vi "TEST - Get Array Element TD.vi"(8 "error in (no error)":errorcluster) -> (0 "error out":errorcluster, 2 "pass":bool)   [LabVIEW 2020, in "test_openg_array.lvlib"]
uses:
  source/library/Type Descriptor.ctl
  test_openg_array.lvlib
  <userlib>/_OpenG.lib/error/error.llb/openg_error.lvlib
  source/library/openg_variant.lvlib
panel:
  out "Failures":T2(array[cluster])
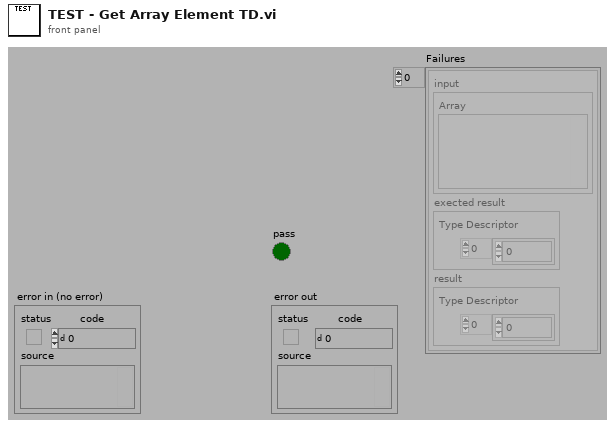
[diagram p1: front panel]
types:
  T1 = typedef "openg_variant.lvlib/Type Descriptor.ctl" = i16[]
  T2 = cluster{"input":cluster{"Array":variant}, "exected result":cluster{"Type Descriptor":T1}, "result":cluster{"Type Descriptor":T1}}[]
  T3 = cluster{"input":cluster{"Array":variant}, "exected result":cluster{"Type Descriptor":T1}, "result":cluster{"Type Descriptor":T1}}
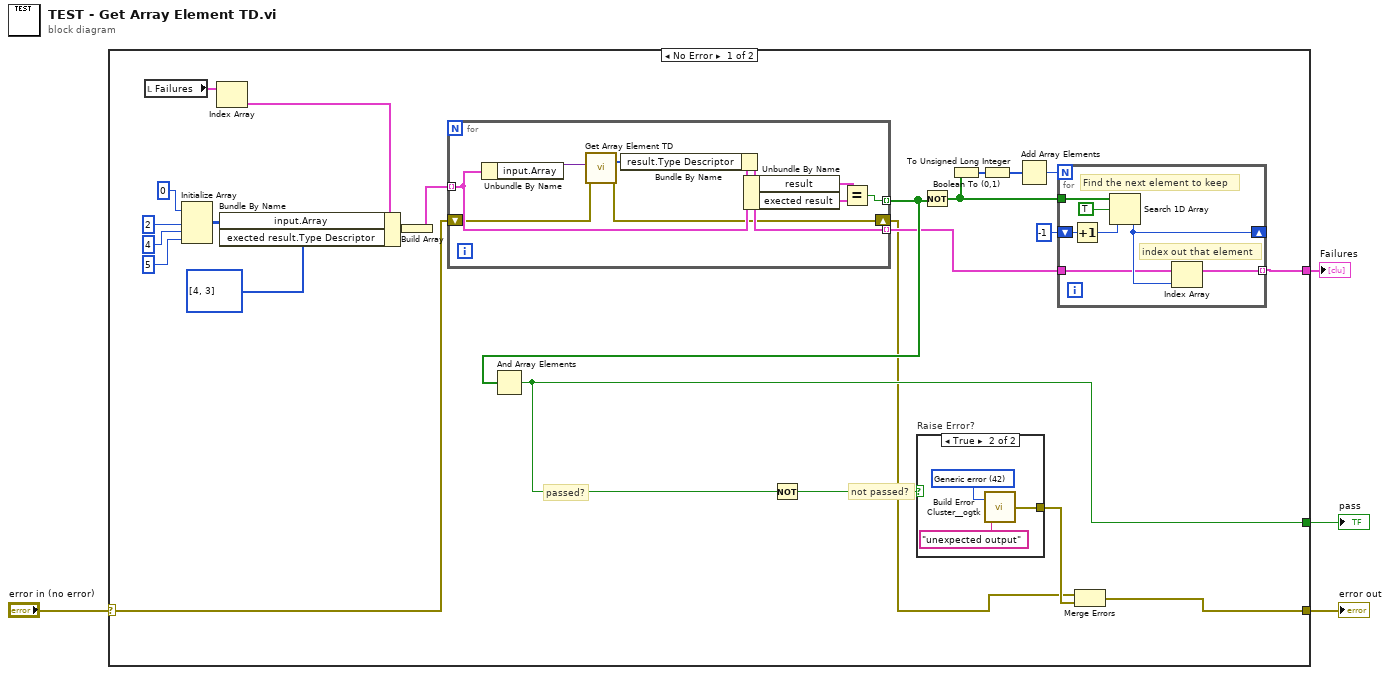
[diagram p0: block diagram]
diagram:
  n1 = case shown="No Error" "error in (no error)" {
    selector: "error in (no error)" -> [w14 w48]
    tunnel: [w25 _] -> w4
    tunnel: [w28 w48] -> w2
    tunnel: [w17 _] -> w1
    frame No Error {
      # "not passed?"
      # "passed?"
      n2 = local read "Failures"() -> (w12:T2)
      n3 = Initialize Array(0, u32 2 ("Numeric"), 4 ("Numeric"), 5 ("Numeric")) -> (w8:i32[][][])
      n4 = Index Array(array=w12) -> (element=w7:T3)  [unwired: 1 in]
      n5 = Bundle By Name(cluster=w7, "input.Array"=w8, "exected result.Type Descriptor"=T1 [4, 3] ("Type Descriptor")) -> (w16:T3)
      n6 = Build Array(w16) -> (w15:T2)
      n7 = for {
        tunnel: w15 -> [w43] mode=indexing
        tunnel: [w44] -> w19 mode=indexing
        tunnel: [w42] -> w18 mode=indexing
        shift-right: [w36] -> w13
        shift-left: w14 -> [w37]
        n8 = Unbundle By Name(w43) -> ("input.Array"=w39:variant)
        n9 = call "Get Array Element TD.vi"("error in (no error)"=w37, "Array"=w39) -> ("error out"=w36:errorcluster, "Type Descriptor"=w38:T1)  [unwired: 8 in]
        n10 = Bundle By Name(cluster=w43, "result.Type Descriptor"=w38) -> (w42:T3)
        n11 = Unbundle By Name(w42) -> ("result"=w41:cluster{"Type Descriptor":T1}, "exected result"=w40:cluster{"Type Descriptor":T1})
        n12 = Equal?(x=w41, y=w40) -> (x = y?=w44:bool)
      }
      n13 = And Array Elements(Boolean array=w19) -> (logical AND=w25:bool)
      n14 = Not(x=w25) -> (.not. x?=w26:bool)
      n15 = case "Raise Error?" shown="True" w26 {
        tunnel: [_ w45] -> w27
        frame False {
        }
        frame True {
          w46 = 42 items=["No error", "Argument error", "Memory is full", "Out of zone", "End of file", "File already open", "Generic file I/O error", "File not found", "File permission error", "Disk is full", "Duplicate path", "Too many files open", "System feature not enabled", "Resource file not found", "Cannot add resource", "Resource not found", "Image not found", "Image memory error", "Pen does not exist", "Config type invalid", "Config token not found", "Config parse error", "Config memory error", "Bad external code format", "Bad external code offset", "External code not present", "Null window", "Destroy window error", "Null menu", "Print aborted", "Bad print record", "Print driver error", "Windows error during printing", "Memory error during printing", "Print dialog error", "Generic print error", "Invalid device refnum", "Device not found", "Device parameter error", "Device unit error", "Cannot open device", "Device call aborted", "Generic error", "Cancelled by user", "Object ID too low", "Object ID too high", "Object not in heap", "Unknown heap", "Unknown object (invalid DefProc)", "Unknown object (DefProc not in table)", "Message out of range", "Invalid (null) method", "Unknown message", "Manager call not supported", "Bad address", "Network operation in progress", "Network operation timed out", "Connection is busy", "Network attribute not supported", "Network error", "Address in use", "System out of memory", "Connection aborted", "Connection refused", "Not connected", "Already connected", "Connection closed", "Initialization error (interapplication manager)", "Bad occurrence", "Wait on unbound occurrence handler", "Occurrence queue overflow", "Datalog type conflict", "Unused", "Unrecognized type (interapplication manager)", "Memory corrupt", "Failed to make temporary DLL", "Old CIN version", "Drag socket not found", "Failed to load drop-object", "Failed to register OLE object", "Failed to release OLE object", "Format specifier type mismatch", "Unknown format specifier", "Too few format specifiers", "Too many format specifiers", "Scan failed", "Newer CIN version", "Error converting to variant", "Runtime menu error", "Password tampered", "Variant attribute not found", "Incompatible variant data type", "Event data is not available", "Event Store is not present", "Occurrence is not found", "Event Queue is not created", "Event info is not available", "Refnum passed is NULL", "Error retrieving Class GUID", "Error retrieving CoClass GUID", "Error retrieving TypeLib GUID.", "Bad built application magic bytes.", "Specific driver is different from the specific driver associated with the Logical Name.", "There is no session opened to the class driver.", "Max Error", "MAX - Error with config objects", "MAX - Error loading configuration", "MAX - Group not supported"]
          n16 = call <userlib>:"Build Error Cluster__ogtk.vi"("String to Prepend to source (\"\")"="unexpected output" ("String to Prepend to source (\"\")"), "code"=w46) -> ("error out"=w45:errorcluster)
        }
      }
      n17 = Not(x=w19) -> (.not. x?=w21:bool[])
      n18 = Boolean To (0,1)(Boolean=w21) -> (0, 1=w22:i16[])
      n19 = To Unsigned Long Integer(number=w22) -> (unsigned 32bit integer=w20:u32[])
      n20 = Add Array Elements(numeric array=w20) -> (sum=w23:u32)
      n21 = for {
        N: w23 -> [_]
        tunnel: w18 -> [w31]
        tunnel: w21 -> [w35]
        shift-right: [w32] -> _
        shift-left: -1 ("start index (0)") -> [w33]
        tunnel: [w30] -> w17 mode=indexing
        # "index out that element"
        # "Find the next element to keep"
        n22 = Increment(x=w33) -> (x+1=w29:i32)
        n23 = Search 1D Array(1D array=w35, element=TRUE, start index (0)=w29) -> (index of element=w32:i32)
        n24 = Index Array(array=w31, index=w32) -> (element=w30:T3)
      }
      n25 = Merge Errors(w13, w27) -> (w28:errorcluster)
    }
    frame Error {
    }
  }
  "pass" <- w4
  "error out" <- w2
  "Failures" <- w1
